vi "Test Migrate v1 Data.vi"(8 "error in (no error)":errorcluster, 10 "Work Folder":path, 11 "Test Data Folder":path) -> (0 "error out":errorcluster, 2 "Report":string, 3 "Passed":bool)   [LabVIEW 2024]
doc: "Migrates a COPY of the version-1 data (Test Data\\v1) with Migrate v1 Data.vi and checks the result: 17 entries over 2025-07 to 2025-10, the projects TimeTracker, Test Project and Test plus an inactive Default project, the Default tasks moved to Settings.ini, the inactive task Test under Test Project, and a second run that does nothing.\n\nInputs: Test Data Folder holds the source copies (Samples, v1); each run works in a new case folder under Work Folder. Passed is TRUE when every check passed and no error occurred; Report lists every check.\n\nGenerated by: Claude"
uses:
  Storage/Time Entry Store-INI/Time Entry Store-INI.lvclass
  Storage/Project Store-INI/Project Store-INI.lvclass
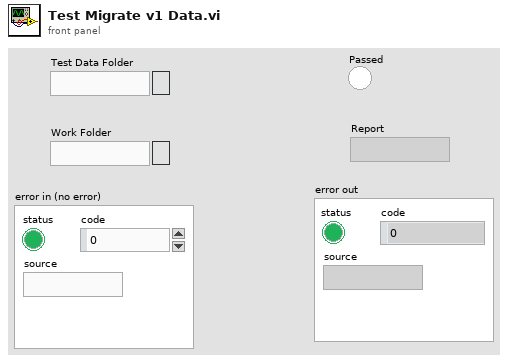
[diagram p1: front panel]
types:
  T1 = typedef "Time Entry List.ctl" = T2[]
  T2 = typedef "Time Entry.ctl" = cluster{"ID":string, "Project ID":string, "Task ID":string, "Start Time":timestamp, "End Time":timestamp, "Description":string}
  T3 = typedef "Project List.ctl" = T4[]
  T4 = typedef "Project.ctl" = cluster{"ID":string, "Name":string, "Active":bool, "Sort Order":i32}
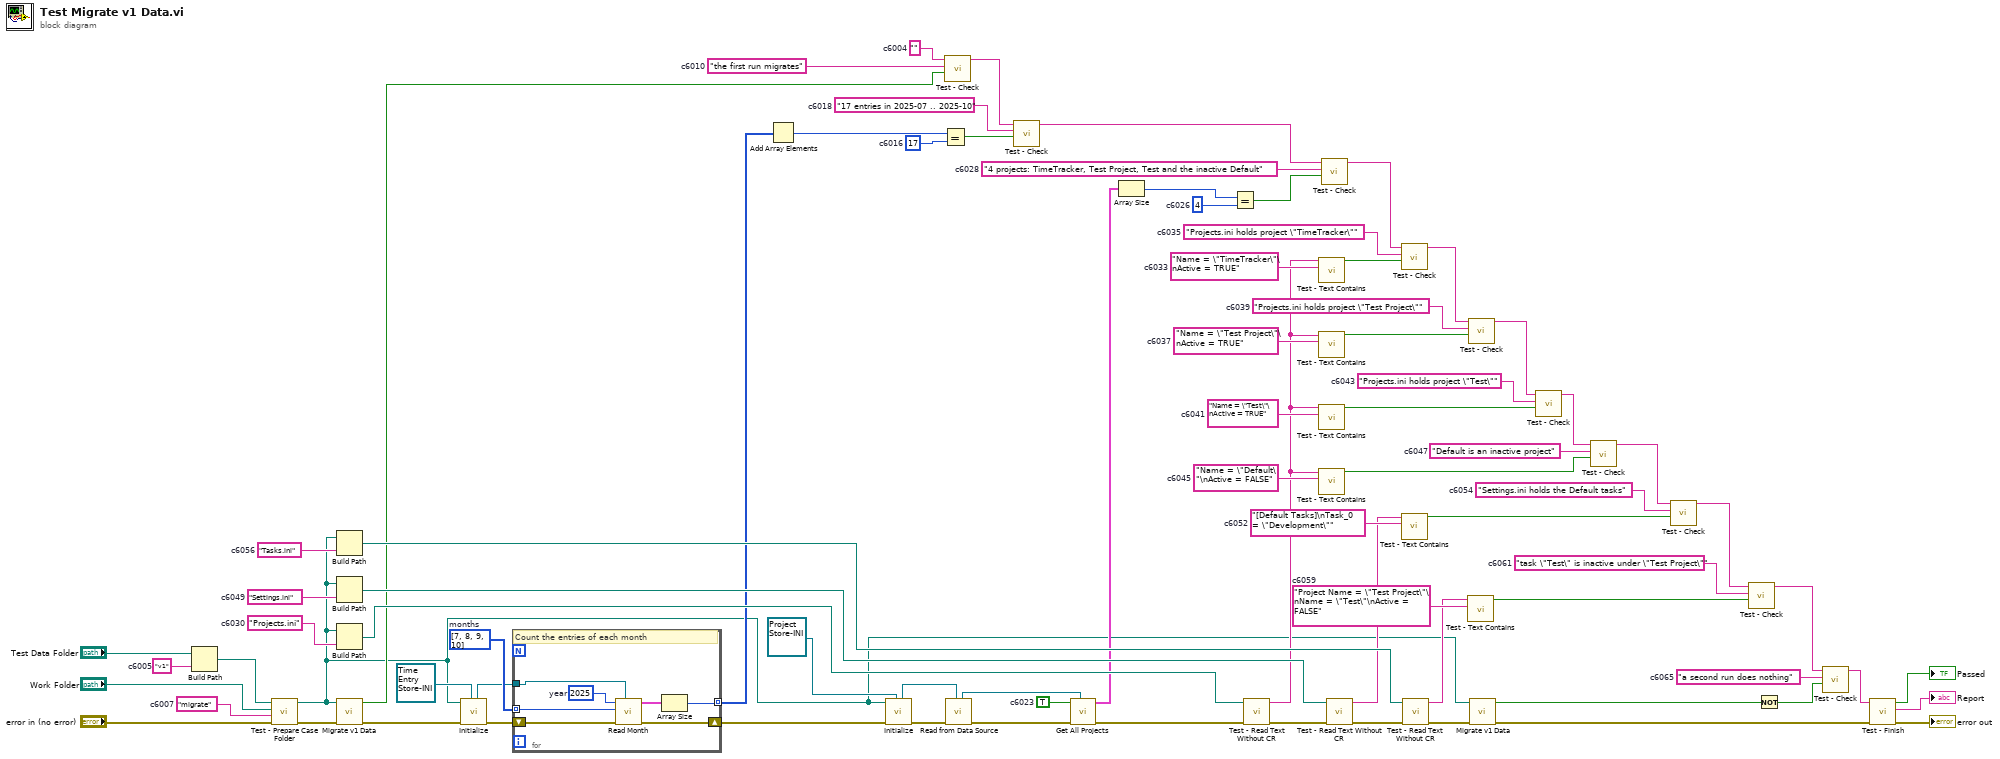
[diagram p0: block diagram]
diagram:
  w77 = "a second run does nothing"  # c6065
  w72 = "task \"Test\" is inactive under \"Test Project\""  # c6061
  w70 = "Project Name = \"Test Project\"\nName = \"Test\"\nActive = FALSE"  # c6059
  w66 = "Tasks.ini"  # c6056
  w64 = "Settings.ini holds the Default tasks"  # c6054
  w62 = "[Default Tasks]\nTask_0 = \"Development\""  # c6052
  w58 = "Settings.ini"  # c6049
  w56 = "Default is an inactive project"  # c6047
  w54 = "Name = \"Default\"\nActive = FALSE"  # c6045
  w52 = "Projects.ini holds project \"Test\""  # c6043
  w50 = "Name = \"Test\"\nActive = TRUE"  # c6041
  w48 = "Projects.ini holds project \"Test Project\""  # c6039
  w46 = "Name = \"Test Project\"\nActive = TRUE"  # c6037
  w44 = "Projects.ini holds project \"TimeTracker\""  # c6035
  w42 = "Name = \"TimeTracker\"\nActive = TRUE"  # c6033
  w38 = "Projects.ini"  # c6030
  w36 = "4 projects: TimeTracker, Test Project, Test and the inactive Default"  # c6028
  w34 = 4  # c6026
  w30 = TRUE  # c6023
  w23 = "17 entries in 2025-07 .. 2025-10"  # c6018
  w21 = 17  # c6016
  w17 = i32[] [7, 8, 9, 10]  # months
  w12 = "the first run migrates"  # c6010
  w7 = "migrate"  # c6007
  w5 = "v1"  # c6005
  w4 = ""  # c6004
  n1 = Build Path(base path="Test Data Folder", name or relative path=w5) -> (appended path=w6:path)
  n2 = call "Test - Prepare Case Folder.vi"("error in (no error)"="error in (no error)", "Case Name"=w7, "Work Folder"="Work Folder", "Source Folder"=w6) -> ("error out"=w9:errorcluster, "Case Folder"=w8:path)  [unwired: 6 in]
  n3 = Build Path(base path=w8, name or relative path=w66) -> (appended path=w67:path)
  n4 = Build Path(base path=w8, name or relative path=w58) -> (appended path=w59:path)
  n5 = Build Path(base path=w8, name or relative path=w38) -> (appended path=w39:path)
  n6 = call "Migrate v1 Data.vi"("error in (no error)"=w9, "Data Folder"=w8) -> ("error out"=w11:errorcluster, "migrated?"=w10:bool)  [unwired: 8 in]
  n7 = call-dynamic "Initialize.vi"("Time Entry Store in"=refnum<class "Time Entry Store-INI.lvclass"> refnum ("Time Entry Store-INI"), "error in (no error)"=w11, "Data Folder"=w8) -> ("error out"=w16:errorcluster, "Time Entry Store out"=w15:refnum<class "Time Entry Store-INI.lvclass">)  [unwired: 7 in]
  n8 = for {
    tunnel: w17 -> [w82] mode=indexing
    tunnel: w15 -> [w83]
    shift-right: [w86] -> w18
    shift-left: w16 -> [w85]
    tunnel: [w88] -> w19 mode=indexing
    w84 = 2025  # year
    # "Count the entries of each month"
    n9 = call-dynamic "Read Month.vi"("Time Entry Store in"=w83, "error in (no error)"=w85, "Month"=w82, "Year"=w84) -> ("error out"=w86:errorcluster, "Time Entries"=w87:T1)  [unwired: 5 in, 1 out]
    n10 = Array Size(array=w87) -> (size(s)=w88:i32)
  }
  n11 = Add Array Elements(numeric array=w19) -> (sum=w20:i32)
  n12 = call-dynamic "Initialize.vi"("Project Store in"=refnum<class "Project Store-INI.lvclass"> refnum ("Project Store-INI"), "error in (no error)"=w18, "Data Folder"=w8) -> ("error out"=w27:errorcluster, "Project Store out"=w26:refnum<class "Project Store-INI.lvclass">)  [unwired: 7 in]
  n13 = Equal?(x=w20, y=w21) -> (x = y?=w22:bool)
  n14 = call "Test - Check.vi"("Condition"=w10, "Check Name"=w12, "Report in"=w4) -> ("Report out"=w13:string)  [unwired: 7 in, 1 out]
  n15 = call-dynamic "Read from Data Source.vi"("Project Store in"=w26, "error in (no error)"=w27) -> ("error out"=w29:errorcluster, "Project Store out"=w28:refnum<class "Project Store-INI.lvclass">)  [unwired: 8 in]
  n16 = call "Test - Check.vi"("Condition"=w22, "Check Name"=w23, "Report in"=w13) -> ("Report out"=w24:string)  [unwired: 7 in, 1 out]
  n17 = call-dynamic "Get All Projects.vi"("Project Store in"=w28, "error in (no error)"=w29, "include inactive?"=w30) -> ("error out"=w32:errorcluster, "Projects"=w31:T3)  [unwired: 6 in, 1 out]
  n18 = Array Size(array=w31) -> (size(s)=w33:i32)
  n19 = Equal?(x=w33, y=w34) -> (x = y?=w35:bool)
  n20 = call "Test - Read Text Without CR.vi"("error in (no error)"=w32, "File"=w39) -> ("error out"=w41:errorcluster, "Text"=w40:string)  [unwired: 8 in]
  n21 = call "Test - Text Contains.vi"("Search Text"=w42, "Text"=w40) -> ("Contains?"=w43:bool)  [unwired: 8 in, 1 out]
  n22 = call "Test - Text Contains.vi"("Search Text"=w46, "Text"=w40) -> ("Contains?"=w47:bool)  [unwired: 8 in, 1 out]
  n23 = call "Test - Text Contains.vi"("Search Text"=w50, "Text"=w40) -> ("Contains?"=w51:bool)  [unwired: 8 in, 1 out]
  n24 = call "Test - Text Contains.vi"("Search Text"=w54, "Text"=w40) -> ("Contains?"=w55:bool)  [unwired: 8 in, 1 out]
  n25 = call "Test - Check.vi"("Condition"=w35, "Check Name"=w36, "Report in"=w24) -> ("Report out"=w37:string)  [unwired: 7 in, 1 out]
  n26 = call "Test - Read Text Without CR.vi"("error in (no error)"=w41, "File"=w59) -> ("error out"=w61:errorcluster, "Text"=w60:string)  [unwired: 8 in]
  n27 = call "Test - Check.vi"("Condition"=w43, "Check Name"=w44, "Report in"=w37) -> ("Report out"=w45:string)  [unwired: 7 in, 1 out]
  n28 = call "Test - Text Contains.vi"("Search Text"=w62, "Text"=w60) -> ("Contains?"=w63:bool)  [unwired: 8 in, 1 out]
  n29 = call "Test - Read Text Without CR.vi"("error in (no error)"=w61, "File"=w67) -> ("error out"=w69:errorcluster, "Text"=w68:string)  [unwired: 8 in]
  n30 = call "Test - Text Contains.vi"("Search Text"=w70, "Text"=w68) -> ("Contains?"=w71:bool)  [unwired: 8 in, 1 out]
  n31 = call "Test - Check.vi"("Condition"=w47, "Check Name"=w48, "Report in"=w45) -> ("Report out"=w49:string)  [unwired: 7 in, 1 out]
  n32 = call "Migrate v1 Data.vi"("error in (no error)"=w69, "Data Folder"=w8) -> ("error out"=w75:errorcluster, "migrated?"=w74:bool)  [unwired: 8 in]
  n33 = call "Test - Check.vi"("Condition"=w51, "Check Name"=w52, "Report in"=w49) -> ("Report out"=w53:string)  [unwired: 7 in, 1 out]
  n34 = call "Test - Check.vi"("Condition"=w55, "Check Name"=w56, "Report in"=w53) -> ("Report out"=w57:string)  [unwired: 7 in, 1 out]
  n35 = call "Test - Check.vi"("Condition"=w63, "Check Name"=w64, "Report in"=w57) -> ("Report out"=w65:string)  [unwired: 7 in, 1 out]
  n36 = call "Test - Check.vi"("Condition"=w71, "Check Name"=w72, "Report in"=w65) -> ("Report out"=w73:string)  [unwired: 7 in, 1 out]
  n37 = Not(x=w74) -> (.not. x?=w76:bool)
  n38 = call "Test - Check.vi"("Condition"=w76, "Check Name"=w77, "Report in"=w73) -> ("Report out"=w78:string)  [unwired: 7 in, 1 out]
  n39 = call "Test - Finish.vi"("error in (no error)"=w75, "Report"=w78) -> ("error out"=→"error out":errorcluster, "Report out"=→"Report":string, "Passed"=→"Passed":bool)  [unwired: 7 in]
